vi "Build CalcExpress Deployment.vi"() -> ()   [LabVIEW 2021]
doc: "::: CalcExpress Toolkit :::\nCopyright (c) 2000-2026 Konstantin Shifershteyn. All rights reserved."
panel:
  in  "Preserve deploy for the current LabVIEW version":bool=TRUE
  out "Excluded files":string
  in  "Exclude undesired paths":bool=TRUE caption="Exclude undesired files & folders"
  # "This VI generates CalcExpress deployment, which is then used for creating a .VIP package."
  # "Before starting this VI, it is strongly recommended to close all VIs that use CalcExpress VIs."
  # "Run this VI to generate CalcExpress deployments, which are saved in the /__Deploy/ folder.\nThe deployment VIs are saved for both the running LabVIEW version and LabVIEW 2014. Both deployments\ninclude the necessary toolkit VIs and assets, and are ready for further distribution.\n\nOptionally, after the deployment for LabVIEW 2014 is built, it is recommended (but not required) to update\nthe DLL linking for the Call Library Function Nodes (CLFN) in that deployment. To do this, open and run\n/__Deploy/Update CLFN in LV2014 Deploy.vi  using  LabVIEW 2014.\n\nBUILD  .VIP  PACKAGE\n\nTo build the CalcExpress distribution package (.VIP), open the CalcExpress (LV2014).vipb file\nin the VIPM Package Builder. This file uses the deployment for LabVIEW 2014 as the source."
  # "CalcExpress Toolkit\nCopyright (c) 2000-2026 Konstantin Shifershteyn"
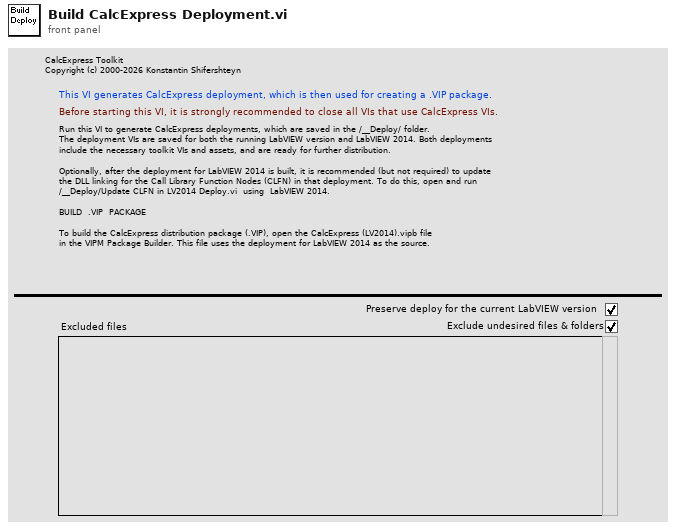
[diagram p1: front panel]
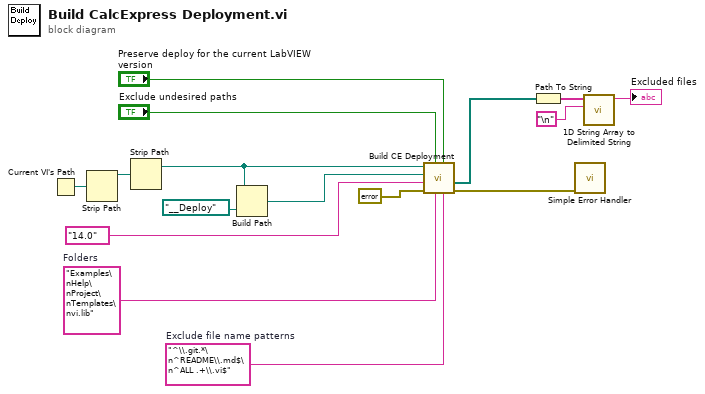
[diagram p0: block diagram]
diagram:
  w10 = "^\\.git.*\n^README\\.md$\n^ALL .+\\.vi$"  # Exclude file name patterns
  w16 = "Examples\nHelp\nProject\nTemplates\nvi.lib"  # Folders
  n1 = Current VI's Path() -> (path=w7:path)
  n2 = Strip Path(path=w7) -> (stripped path=w8:path)  [unwired: 1 out]
  n3 = Strip Path(path=w8) -> (stripped path=w5:path)  [unwired: 1 out]
  n4 = Build Path(base path=w5, name or relative path=path "__Deploy" ("Target Dir")) -> (appended path=w3:path)
  n5 = call "Build CE Deployment.vi"("Exclude file name patterns"=w10, "preserve current version code (T)"="Preserve deploy for the current LabVIEW version", "Folders"=w16, "Exclude undesired paths (T)"="Exclude undesired paths", "error in"=errorcluster {"status"=FALSE, "code"=0, "source"=""}, "LV Version"="14.0", "Target Dir"=w3, "Source Dir"=w5) -> ("error out"=w6:errorcluster, "Excluded Paths"=w14:path[])  [unwired: 2 out]
  n6 = Path To String(path=w14) -> (string=w13:string[])
  n7 = call <vilib>:"Simple Error Handler.vi"("error in (no error)"=w6) -> ()  [unwired: 4 in, 5 out]
  n8 = call <vilib>:"1D String Array to Delimited String.vi"("delimiter"="\n", "string array"=w13) -> ("delimited string"=→"Excluded files":string)  [unwired: 9 in]
